vi "Divide float (multiple).vi"(8 "error in (no error)":errorcluster, 9 "y (1)":dbl=1.0, 10 "x (1)":dbl=1.0, 11 "XY-data":cluster{"X-array":dbl[], "Y-array":dbl[]}[](array[cluster]) {"Y-array" format="%.2p"; "X-array" format="%.2p"}) -> (0 "error out":errorcluster, 3 "XY-data out":cluster{"X-array":dbl[], "Y-array":dbl[]}[](array[cluster]) {"Y-array" format="%.2p"; "X-array" format="%.2p"})   [LabVIEW 2019, in "xy_utilities.lvlib"]
doc: "Divide the x array of <b>XY-data</b> by <b>x</b>\nDivide the y array of <b>XY-data</b> by <b>y</b>\n\nWire data to the data input to determine the polymorphic instance to use or manually select the instance."
uses:
  xy_utilities.lvlib
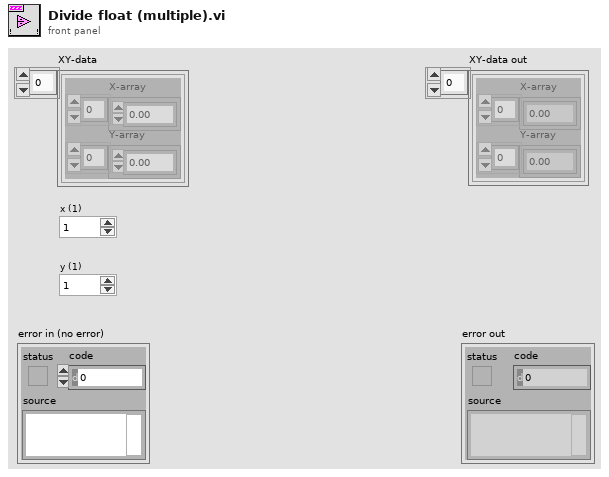
[diagram p1: front panel]
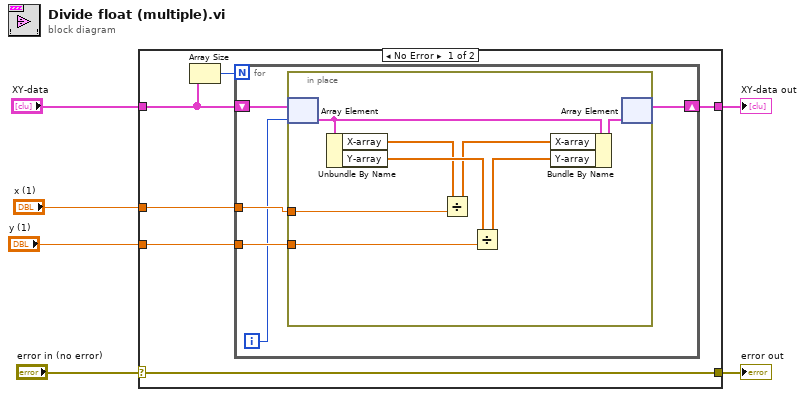
[diagram p0: block diagram]
diagram:
  n1 = case shown="No Error" "error in (no error)" {
    selector: "error in (no error)" -> [w12 w27]
    tunnel: [w12 w27] -> w5
    tunnel: "XY-data" -> [w7 w26]
    tunnel: [w11 w26] -> w3
    tunnel: "y (1)" -> [w10 _]
    tunnel: "x (1)" -> [w9 _]
    frame No Error {
      n2 = Array Size(array=w7) -> (size(s)=w8:i32)
      n3 = for {
        N: w8 -> [_]
        tunnel: w10 -> [w17]
        tunnel: w9 -> [w16]
        shift-right: [w13] -> w11
        shift-left: w7 -> [w15]
        i -> [w14]
        n4 = in-place {
          in-place-border: w17 -> [w25]
          in-place-border: w16 -> [w20]
          n5 = in-place-array #1(w15, w14) -> (w19:cluster{"X-array":dbl[], "Y-array":dbl[]})
          n6 = Unbundle By Name(w19) -> ("X-array"=w21:dbl[], "Y-array"=w24:dbl[])
          n7 = Divide(x=w21, y=w20) -> (x/y=w22:dbl[])
          n8 = Divide(x=w24, y=w25) -> (x/y=w23:dbl[])
          n9 = Bundle By Name(cluster=w19, "X-array"=w22, "Y-array"=w23) -> (w18:cluster{"X-array":dbl[], "Y-array":dbl[]})
          n10 = in-place-array #1(w18) -> (w13:cluster{"X-array":dbl[], "Y-array":dbl[]}[])  [unwired: 1 out]
        }
      }
    }
    frame Error {
    }
  }
  "error out" <- w5
  "XY-data out" <- w3
